vi "libssh2_hostkey_hash.vi"(8 "error in (no error)":errorcluster, 10 "hash type":T1=enum."SHA1", 11 "session":T2) -> (0 "error out":errorcluster, 2 "hash":u8[](array[numeric]))   [LabVIEW 2017, in "libssh2.lvlib"]
doc: "Get the hash of the remote host's public key."
uses:
  libssh2.lvlib
  Session Refnum.ctl
  Host Key Hash Type.ctl
  Not A Session.vi
  <vilib>/Utility/error.llb/Error Cluster From Error Code.vi
  Global Settings.vi
  Read Session Refnum.vi
  <vilib>/Utility/semaphor.llb/Acquire Semaphore.vi
  <vilib>/Utility/semaphor.llb/Release Semaphore.vi
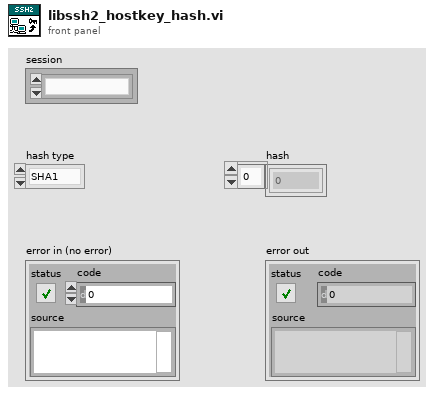
[diagram p1: front panel]
types:
  T1 = typedef "libssh2.lvlib/Host Key Hash Type.ctl" = enum16{"MD5", "SHA1", "SHA256"}
  T2 = typedef "libssh2.lvlib/Session Refnum.ctl" = refnum<k1>
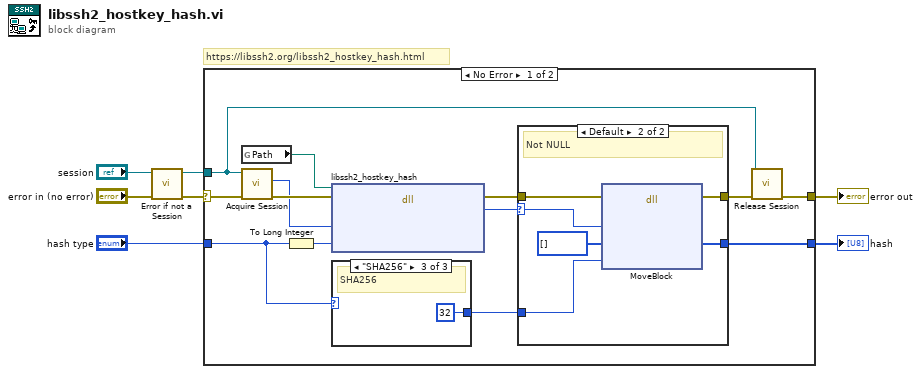
[diagram p0: block diagram]
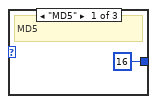
[diagram p3: hidden frame]
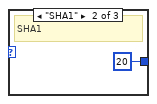
[diagram p4: hidden frame]
diagram:
  # "https://libssh2.org/libssh2_hostkey_hash.html"
  n1 = call "Error if not a Session.vi"("error in (no error)"="error in (no error)", "session"="session") -> ("error out"=w3:errorcluster, "session out"=w1:T2)  [unwired: 8 in]
  n2 = case shown="No Error" w3 {
    selector: w3 -> [w20 w31]
    tunnel: "hash type" -> [w18 _]
    tunnel: [w9 w31] -> w6
    tunnel: w1 -> [w8 _]
    tunnel: [w17 _] -> w4
    frame No Error {
      n3 = global read "Global Settings.vi" "Path"() -> (w12:path)
      n4 = call "Acquire Session.vi"("error in (no error)"=w20, "session"=w8) -> ("error out"=w16:errorcluster, "LIBSSH2_SESSION*"=w15:u64)  [unwired: 7 in, 1 out]
      n5 = To Long Integer(number=w18) -> (32bit integer=w10:i32)
      n6 = dll-call lib="?" fn="libssh2_hostkey_hash"(path in=w12, error in=w16, "session"=w15, "hash_type"=w10) -> (error out=w14:errorcluster, "return value"=w11:u64)  [unwired: 3 in, 1 out]
      n7 = case shown="\"SHA256\"" w18 {
        tunnel: [u64 16 ("dimension size") u64 20 ("dimension size") u64 32 ("dimension size")] -> w13
        frame "MD5" {
          # "MD5"
        }
        frame "SHA1" {
          # "SHA1"
        }
        frame "SHA256" {
          # "SHA256"
        }
      }
      n8 = case shown="Default" w11 {
        selector: w11 -> [_ w22]
        tunnel: w14 -> [w21 w27]
        tunnel: [w21 w26] -> w19
        tunnel: w13 -> [_ w24]
        tunnel: [_ w23] -> w17
        frame 0 {
          # "NULL"
        }
        frame Default {
          # "Not NULL"
          n9 = dll-call lib="LabVIEW" fn="MoveBlock"(error in=w27, "ps"=w22, "pd"=u8[] [], "size"=w24) -> (error out=w26:errorcluster, "pd"=w23:u8[])  [unwired: 5 in, 1 out]
        }
      }
      n10 = call "Release Session.vi"("error in (no error)"=w19, "session"=w8) -> ("error out"=w9:errorcluster)  [unwired: 9 in]
    }
    frame Error {
    }
  }
  "error out" <- w6
  "hash" <- w4
